vi "MB Read_Cached.vi"(8 "error in (no error)":errorcluster, 9 "Quantity(1)":u16=1, 10 "Modbus Reference":u32, 11 "MB PLC in":refnum<class "MB PLC Client.lvclass">) -> (0 "error out":errorcluster, 3 "MB PLC out":refnum<class "MB PLC Client.lvclass">)   [LabVIEW 2018, in "MB PLC Client.lvlib" / "MB PLC Client.lvclass"]
uses:
  MB PLC Client.lvclass
  MB PLC Client.lvclass/MB PLC Client.ctl
  <vilib>/Utility/error.llb/Error Cluster From Error Code.vi
  <vilib>/ErrorRing/Error Ring.xnode
  Data/MB Data Block.lvclass
  <vilib>/Plasmionique/MB Master/MB Master.lvlib
  MB PLC Client.lvlib
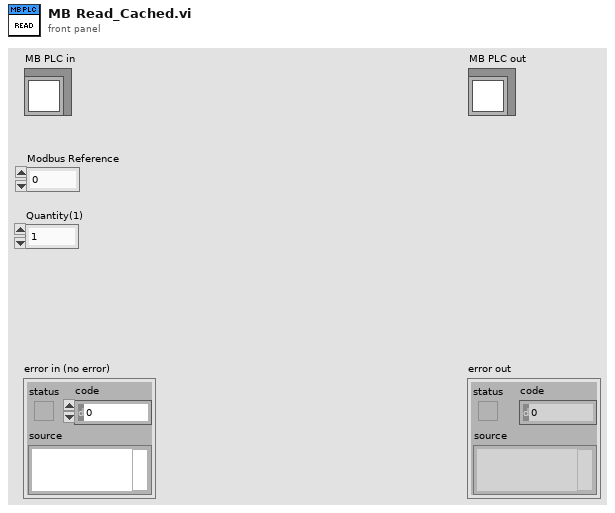
[diagram p1: front panel]
types:
  T1 = typedef "MB PLC Client.lvlib/Reference Types_Enum.ctl" = enum16{"Coil", "Discrete Input", "Input Register", "Holding Register", "Invalid"}
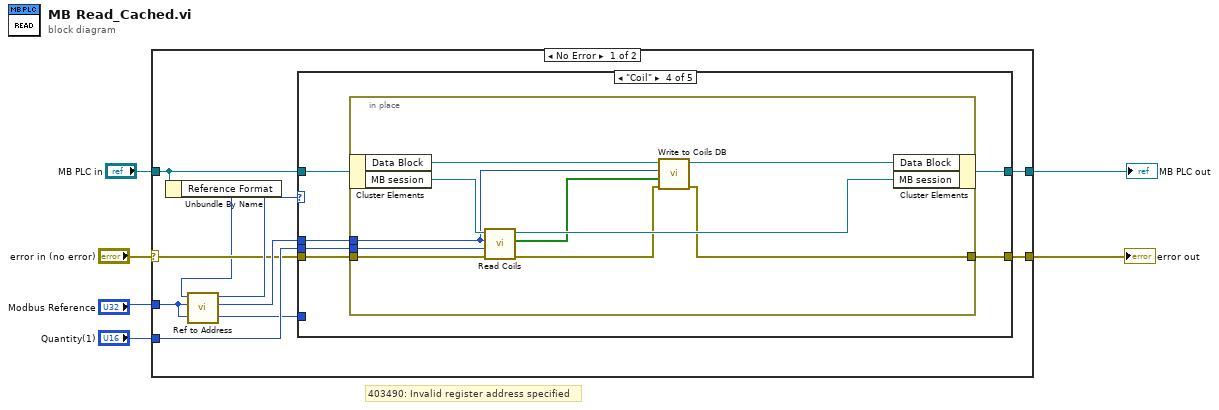
[diagram p0: block diagram]
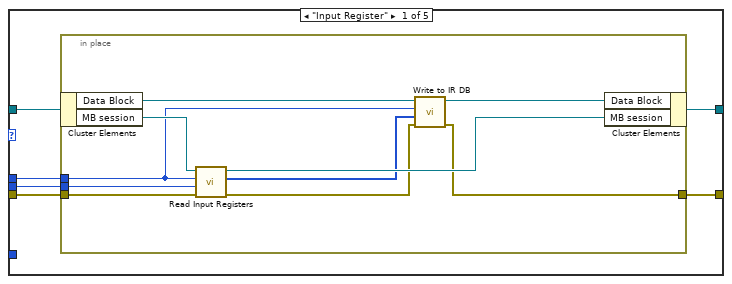
[diagram p2: hidden frame]
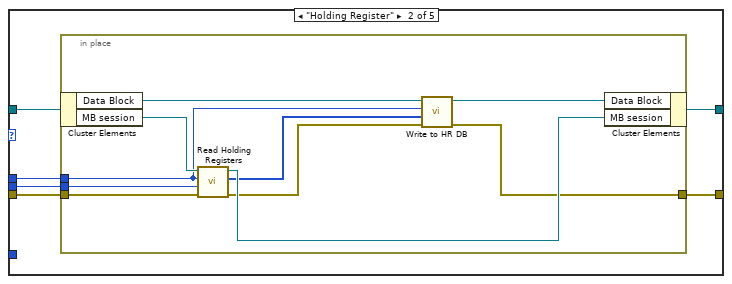
[diagram p3: hidden frame]
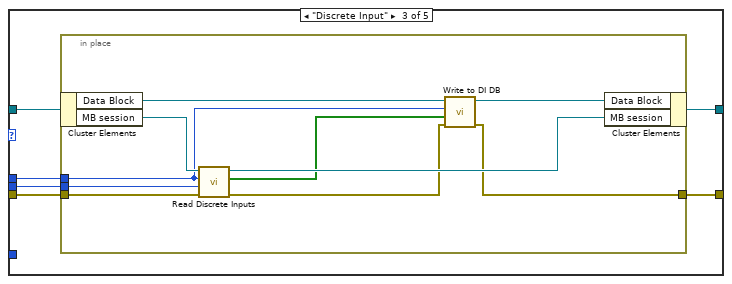
[diagram p4: hidden frame]
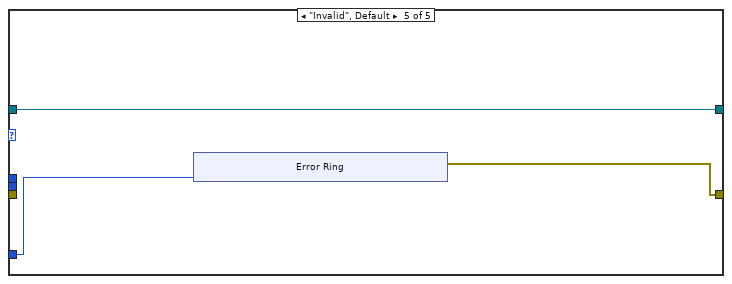
[diagram p5: hidden frame]
diagram:
  # "403490: Invalid register address specified"
  n1 = case shown="No Error" "error in (no error)" {
    selector: "error in (no error)" -> [w10 w90]
    tunnel: [w13 w90] -> w6
    tunnel: "Quantity(1)" -> [w12 _]
    tunnel: "Modbus Reference" -> [w9 _]
    tunnel: "MB PLC in" -> [w8 w91]
    tunnel: [w11 w91] -> w2
    frame No Error {
      n2 = Unbundle By Name(w8) -> ("Reference Format"=w7:u16)
      n3 = call "Ref to Address.vi"("Reference"=w9, "Reference Format"=w7) -> ("Address"=w15:u16, "Reference Type"=w14:T1)  [unwired: 8 in]
      n4 = case shown="\"Coil\"" w14 {
        tunnel: w15 -> [w18 w34 w50 w66 _]
        tunnel: w12 -> [w19 w35 w51 w67 _]
        tunnel: w10 -> [w20 w36 w52 w68 _]
        tunnel: [w21 w37 w53 w69 w80] -> w13
        tunnel: w8 -> [w17 w33 w49 w65 w82]
        tunnel: [w16 w32 w48 w64 w82] -> w11
        tunnel: w9 -> [_ _ _ _ w81]
        frame "Input Register" {
          # "Input Reg"
          n5 = in-place {
            in-place-border: [w24] -> w21
            in-place-border: w20 -> [w31]
            in-place-border: w19 -> [w28]
            in-place-border: w18 -> [w23]
            n6 = in-place-cluster #1(w17) -> ("Data Block"=w27:refnum<class "MB Data Block.lvclass">, "MB session"=w30:refnum<class "MB_Master.lvclass">)
            n7 = call <vilib>:"Read Input Registers.vi"("error in (no error)"=w31, "quantity"=w28, "starting address"=w23, "MB session in"=w30) -> ("error out"=w25:errorcluster, "Registers"=w22:u16[], "MB session out"=w29:refnum<class "MB_Master.lvclass">)  [unwired: 5 in]
            n8 = call-dynamic "Write to IR DB.vi"("error in (no error)"=w25, "Values"=w22, "Modbus Address"=w23, "MB Cache in"=w27) -> ("error out"=w24:errorcluster, "MB Cache out"=w26:refnum<class "MB Data Block.lvclass">)  [unwired: 6 in]
            n9 = in-place-cluster #1("Data Block"=w26, "MB session"=w29) -> (w16:refnum<class "MB PLC Client.lvclass">)
          }
        }
        frame "Holding Register" {
          # "Input Reg"
          n10 = in-place {
            in-place-border: [w38] -> w37
            in-place-border: w36 -> [w47]
            in-place-border: w35 -> [w46]
            in-place-border: w34 -> [w40]
            n11 = in-place-cluster #2(w33) -> ("Data Block"=w43:refnum<class "MB Data Block.lvclass">, "MB session"=w45:refnum<class "MB_Master.lvclass">)
            n12 = call <vilib>:"Read Holding Registers.vi"("error in (no error)"=w47, "quantity"=w46, "starting address"=w40, "MB session in"=w45) -> ("error out"=w39:errorcluster, "Registers"=w41:u16[], "MB session out"=w44:refnum<class "MB_Master.lvclass">)  [unwired: 5 in]
            n13 = call-dynamic "Write to HR DB.vi"("error in (no error)"=w39, "Values"=w41, "Modbus Address"=w40, "MB Cache in"=w43) -> ("error out"=w38:errorcluster, "MB Cache out"=w42:refnum<class "MB Data Block.lvclass">)  [unwired: 6 in]
            n14 = in-place-cluster #2("Data Block"=w42, "MB session"=w44) -> (w32:refnum<class "MB PLC Client.lvclass">)
          }
        }
        frame "Discrete Input" {
          # "Input Reg"
          n15 = in-place {
            in-place-border: [w56] -> w53
            in-place-border: w52 -> [w62]
            in-place-border: w51 -> [w61]
            in-place-border: w50 -> [w54]
            n16 = in-place-cluster #3(w49) -> ("Data Block"=w59:refnum<class "MB Data Block.lvclass">, "MB session"=w63:refnum<class "MB_Master.lvclass">)
            n17 = call <vilib>:"Read Discrete Inputs.vi"("error in (no error)"=w62, "quantity"=w61, "starting address"=w54, "MB session in"=w63) -> ("error out"=w57:errorcluster, "Inputs"=w55:bool[], "MB session out"=w60:refnum<class "MB_Master.lvclass">)  [unwired: 5 in]
            n18 = call-dynamic "Write to DI DB.vi"("error in (no error)"=w57, "Values"=w55, "Modbus Address"=w54, "MB Cache in"=w59) -> ("error out"=w56:errorcluster, "MB Cache out"=w58:refnum<class "MB Data Block.lvclass">)  [unwired: 6 in]
            n19 = in-place-cluster #3("Data Block"=w58, "MB session"=w60) -> (w48:refnum<class "MB PLC Client.lvclass">)
          }
        }
        frame "Coil" {
          # "Input Reg"
          n20 = in-place {
            in-place-border: [w73] -> w69
            in-place-border: w68 -> [w79]
            in-place-border: w67 -> [w78]
            in-place-border: w66 -> [w70]
            n21 = in-place-cluster #4(w65) -> ("Data Block"=w75:refnum<class "MB Data Block.lvclass">, "MB session"=w77:refnum<class "MB_Master.lvclass">)
            n22 = call <vilib>:"Read Coils.vi"("error in (no error)"=w79, "quantity"=w78, "starting address"=w70, "MB session in"=w77) -> ("error out"=w74:errorcluster, "Coils"=w71:bool[], "MB session out"=w76:refnum<class "MB_Master.lvclass">)  [unwired: 5 in]
            n23 = call-dynamic "Write to Coils DB.vi"("error in (no error)"=w74, "Values"=w71, "Modbus Address"=w70, "MB Cache in"=w75) -> ("error out"=w73:errorcluster, "MB Cache out"=w72:refnum<class "MB Data Block.lvclass">)  [unwired: 6 in]
            n24 = in-place-cluster #4("Data Block"=w72, "MB session"=w76) -> (w64:refnum<class "MB PLC Client.lvclass">)
          }
        }
        frame "Invalid", Default {
          # "Invalid"
          n25 = xnode "Error Ring"("parameter 0"=w81) -> ("error out"=w80:errorcluster)
        }
      }
    }
    frame Error {
    }
  }
  "error out" <- w6
  "MB PLC out" <- w2
